vi "Interlock.vi"(8 "error in":errorcluster, 11 "VISA resource name":refnum<visa-resource-name>) -> (0 "error out":errorcluster, 3 "RESULT":bool)   [LabVIEW 2021]
uses:
  HI-POT_Driver/GPT-9800_GSB_L8.5/GPT-9000.lvlib
panel:
  out "Return  the test status":string
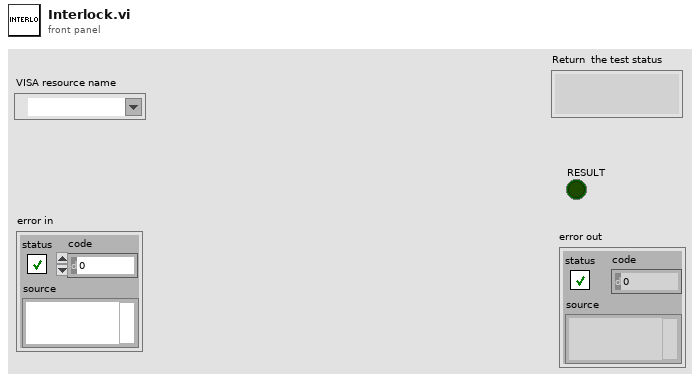
[diagram p1: front panel]
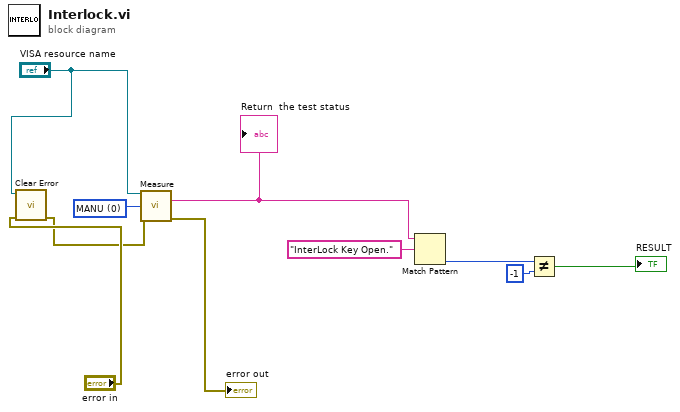
[diagram p0: block diagram]
diagram:
  w7 = u8 0 items=["MANU", "AUTO"] ("Function Mode Numeric")
  n1 = call "Clear Error.vi"("error in (no error)"="error in", "VISA resource name"="VISA resource name") -> ("error out"=w1:errorcluster)  [unwired: 8 in, 1 out]
  n2 = call "Measure.vi"("VISA resource name"="VISA resource name", "Function Mode Numeric"=w7, "error in"=w1) -> ("Return  the test status"=w4:string, "error out"=→"error out":errorcluster)  [unwired: 9 in, 2 out]
  "Return  the test status" <- w4
  n3 = Match Pattern(string=w4, regular expression="InterLock Key Open.") -> (offset past match=w9:i32)  [unwired: 1 in, 3 out]
  n4 = Not Equal?(x=w9, y=-1) -> (x != y?=→"RESULT":bool)
